vi "RemoteVI Frame Rect.vi"(0 "hWnd":u64, 11 "error in":errorcluster) -> (4 "rect":cluster{"x":i32, "y":i32, "w":i32, "h":i32}, 15 "error out":errorcluster)   [LabVIEW 2020, in "RemoteVI.lvlib"]
doc: "Where the FRAME of the window hWnd is on screen - the part of the front panel window that RemoteVI streams: its client area, everything below the title bar and inside the borders. For a LabVIEW front panel that is the menu bar, the toolbar, the panel and its scrollbars: LabVIEW draws its menu bar itself inside the client area (measured on LabVIEW 2025: GetMenu returns NULL and GetMenuBarInfo fails for a panel with the default and with a custom run-time menu bar), and so are the toolbar and the panel scrollbars. rect.x and rect.y are the screen position of the client-area origin (the negative of user32 ScreenToClient applied to the screen point 0,0), rect.w and rect.h its size (user32 GetClientRect). A minimized or vanished window gives w or h 0. Win32 only, no VI Server call, so it works while a popup's modal loop holds LabVIEW's UI thread."
uses:
  RemoteVI.lvlib
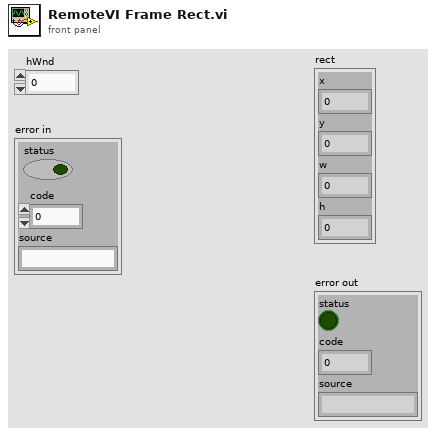
[diagram p1: front panel]
types:
  T1 = cluster{"left":i32, "top":i32, "right":i32, "bottom":i32}
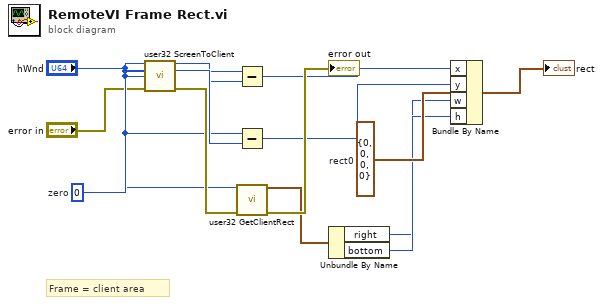
[diagram p0: block diagram]
diagram:
  w13 = cluster{"x":i32, "y":i32, "w":i32, "h":i32} {"x"=0, "y"=0, "w"=0, "h"=0}  # rect0
  w3 = 0  # zero
  # "Frame = client area"
  n1 = call "user32 ScreenToClient.vi"("hWnd"="hWnd", "Screen X"=w3, "Screen Y"=w3, "error in (no error)"="error in") -> ("Client X"=w4:i32, "Client Y"=w5:i32, "error out"=w6:errorcluster)  [unwired: 8 in, 1 out]
  n2 = Subtract(x=w3, y=w4) -> (x-y=w7:i32)
  n3 = Subtract(x=w3, y=w5) -> (x-y=w8:i32)
  n4 = call "user32 GetClientRect.vi"("hWnd"="hWnd", "error in"=w6) -> ("RECT"=w9:T1, "error out"=→"error out":errorcluster)  [unwired: 11 in, 1 out]
  n5 = Unbundle By Name(w9) -> ("right"=w11:i32, "bottom"=w12:i32)
  n6 = Bundle By Name(cluster=w13, "x"=w7, "y"=w8, "w"=w11, "h"=w12) -> (→"rect":cluster{"x":i32, "y":i32, "w":i32, "h":i32})
